vi "Tranfer String to Timestamp.vi"(9 "File Type":T1, 11 "String":string="44568.9754166667") -> (3 "time stamp":timestamp)   [LabVIEW 2020, in "Data Viewer.lvlib"]
uses:
  Data Viewer.lvlib
  File Type--enum.ctl
  <vilib>/Utility/miscctls.llb/LVDateTimeRec.ctl
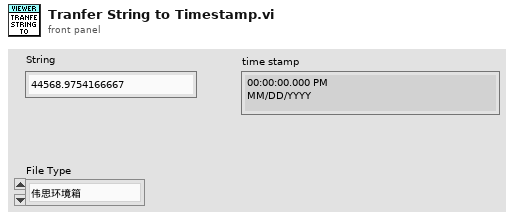
[diagram p1: front panel]
types:
  T1 = typedef "Data Viewer.lvlib/File Type--enum.ctl" = enum16{"伟思环境箱", "增达环境箱", "广五所环境箱", "无纸记录仪", "帕捷SA00339", "记录仪840", "记录仪8400", "记录仪MR888", "*.csv"}
  T2 = typedef "LVDateTimeRec.ctl" = cluster{"fractional second":dbl, "second":i32, "minute":i32, "hour":i32, "day of month":i32, "month":i32, "year":i32, "day of week":i32, "day of year":i32, "DST":i32}
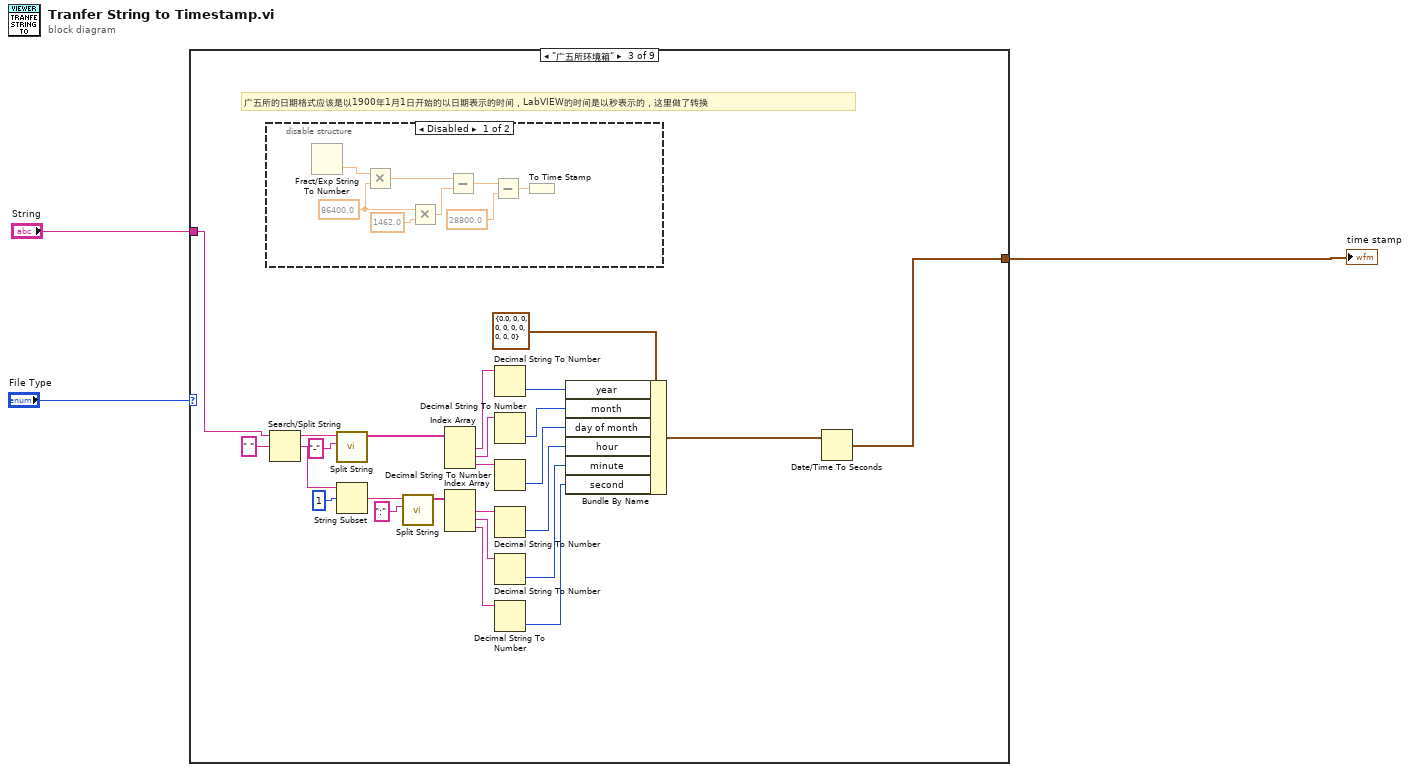
[diagram p0: block diagram]
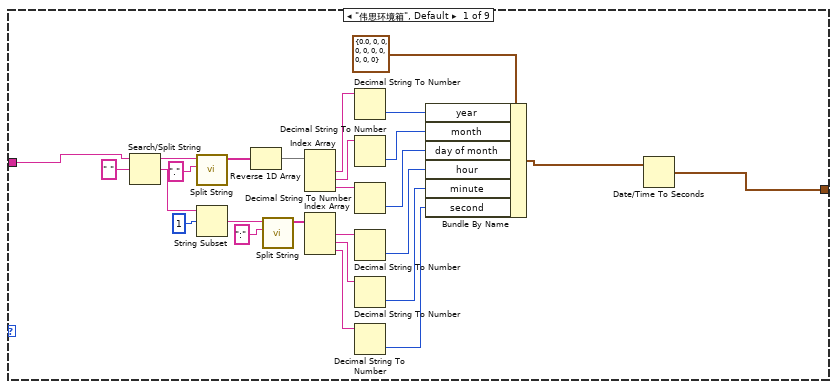
[diagram p2: hidden frame]
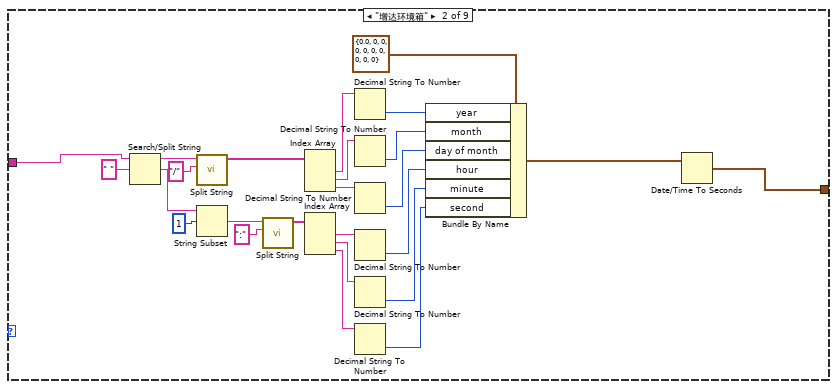
[diagram p3: hidden frame]
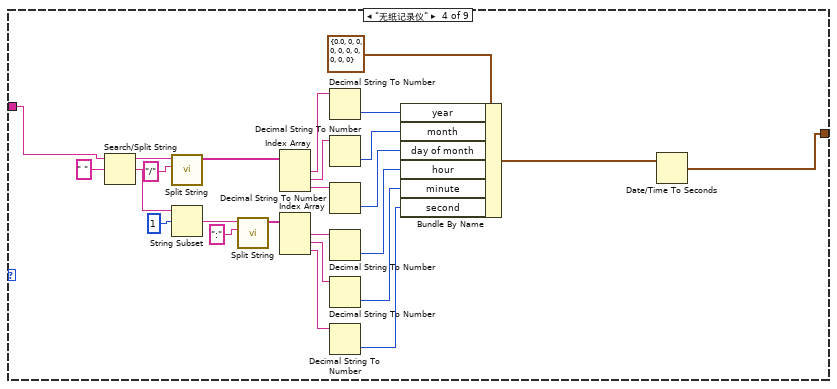
[diagram p5: hidden frame]
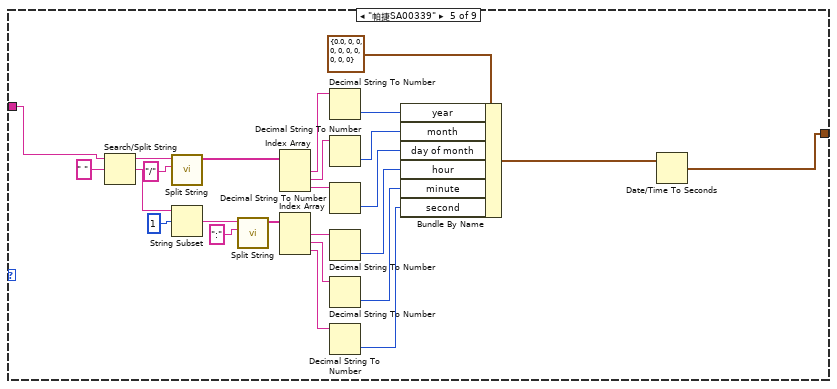
[diagram p6: hidden frame]
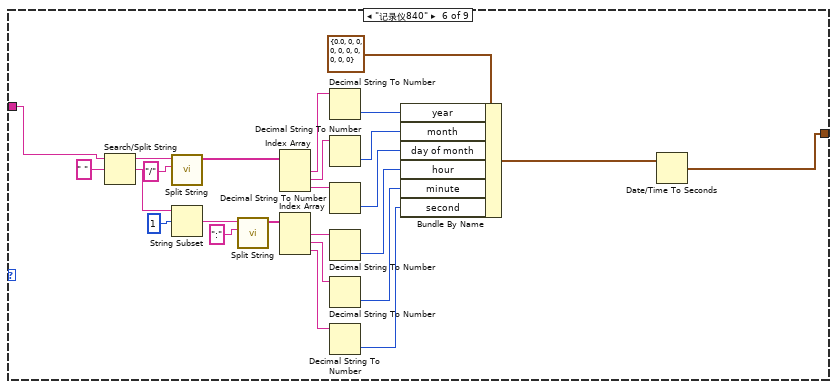
[diagram p7: hidden frame]
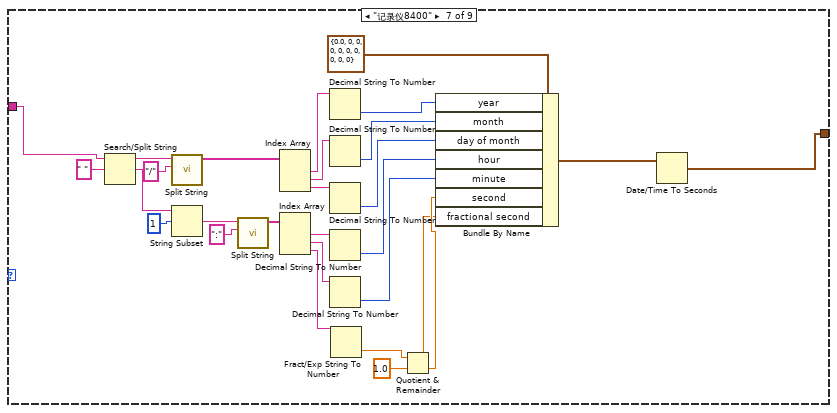
[diagram p8: hidden frame]
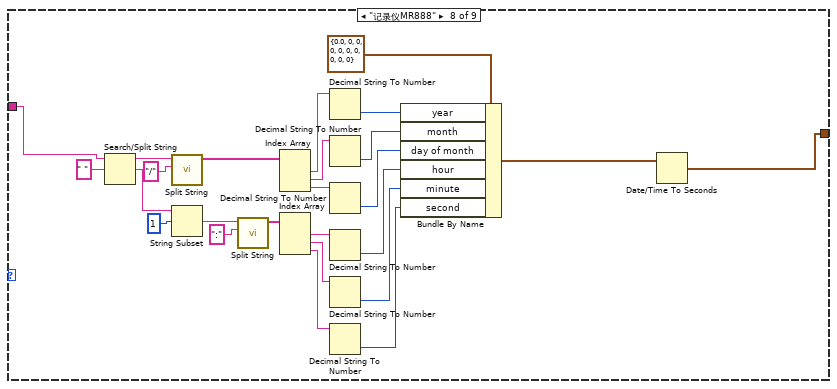
[diagram p9: hidden frame]
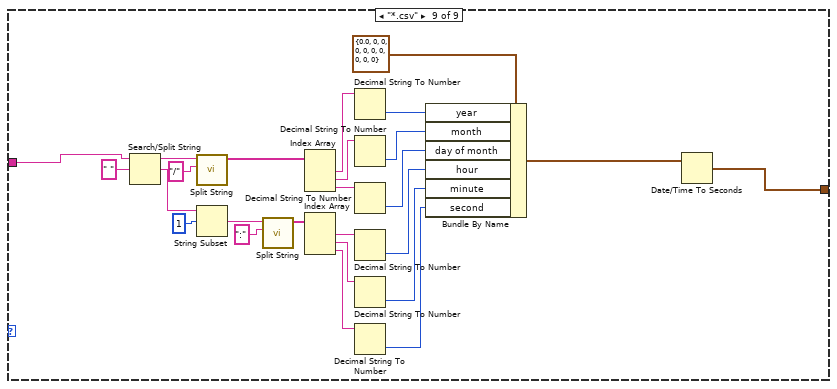
[diagram p10: hidden frame]
diagram:
  n1 = case shown="\"广五所环境箱\"" "File Type" {
    tunnel: "String" -> [w29 w54 w56 w112 w114 w139 w169 w192 w240]
    tunnel: [w4 w30 w55 w111 w113 w138 w168 w191 w216] -> w1
    frame "伟思环境箱", Default {
      n2 = Search/Split String(string=w29, search string/char (-)=" ") -> (substring before match=w22:string, match + rest of string=w27:string)  [unwired: 1 in, 1 out]
      n3 = call "Split String.vi"("分隔字符(;)"=".", "字符串"=w22) -> ("字符串数组"=w20:string[])  [unwired: 8 in, 1 out]
      n4 = String Subset(string=w27, offset (0)=1) -> (substring=w25:string)  [unwired: 1 in]
      n5 = Reverse 1D Array(array=w20) -> (reversed array=w19:string[])
      n6 = call "Split String.vi"("分隔字符(;)"=":", "字符串"=w25) -> ("字符串数组"=w9:string[])  [unwired: 8 in, 1 out]
      n7 = Index Array(array=w19) -> (element #1=w18:string, element #2=w17:string, element #3=w16:string)  [unwired: 3 in]
      n8 = Index Array(array=w9) -> (element #1=w10:string, element #2=w11:string, element #3=w12:string)  [unwired: 3 in]
      n9 = Decimal String To Number(string=w18) -> (number=w15:i32)  [unwired: 2 in, 1 out]
      n10 = Decimal String To Number(string=w17) -> (number=w14:i32)  [unwired: 2 in, 1 out]
      n11 = Decimal String To Number(string=w16) -> (number=w13:i32)  [unwired: 2 in, 1 out]
      n12 = Decimal String To Number(string=w10) -> (number=w7:i32)  [unwired: 2 in, 1 out]
      n13 = Decimal String To Number(string=w11) -> (number=w8:i32)  [unwired: 2 in, 1 out]
      n14 = Decimal String To Number(string=w12) -> (number=w6:i32)  [unwired: 2 in, 1 out]
      n15 = Bundle By Name(cluster=T2 {"fractional second"=0.0, "second"=0, "minute"=0, "hour"=0, "day of month"=0, "month"=0, "year"=0, "day of week"=0, "day of year"=0, "DST"=0} ("date time rec"), "year"=w15, "month"=w14, "day of month"=w13, "hour"=w7, "minute"=w8, "second"=w6) -> (w5:T2)
      n16 = Date/Time To Seconds(2:w5) -> (0:w4:timestamp)  [unwired: 1 in]
    }
    frame "增达环境箱" {
      n17 = Search/Split String(string=w54, search string/char (-)=" ") -> (substring before match=w47:string, match + rest of string=w52:string)  [unwired: 1 in, 1 out]
      n18 = call "Split String.vi"("分隔字符(;)"="/", "字符串"=w47) -> ("字符串数组"=w45:string[])  [unwired: 8 in, 1 out]
      n19 = String Subset(string=w52, offset (0)=1) -> (substring=w50:string)  [unwired: 1 in]
      n20 = call "Split String.vi"("分隔字符(;)"=":", "字符串"=w50) -> ("字符串数组"=w35:string[])  [unwired: 8 in, 1 out]
      n21 = Index Array(array=w45) -> (element #1=w44:string, element #2=w43:string, element #3=w42:string)  [unwired: 3 in]
      n22 = Index Array(array=w35) -> (element #1=w36:string, element #2=w37:string, element #3=w38:string)  [unwired: 3 in]
      n23 = Decimal String To Number(string=w44) -> (number=w41:i32)  [unwired: 2 in, 1 out]
      n24 = Decimal String To Number(string=w43) -> (number=w40:i32)  [unwired: 2 in, 1 out]
      n25 = Decimal String To Number(string=w42) -> (number=w39:i32)  [unwired: 2 in, 1 out]
      n26 = Decimal String To Number(string=w36) -> (number=w33:i32)  [unwired: 2 in, 1 out]
      n27 = Decimal String To Number(string=w37) -> (number=w34:i32)  [unwired: 2 in, 1 out]
      n28 = Decimal String To Number(string=w38) -> (number=w32:i32)  [unwired: 2 in, 1 out]
      n29 = Bundle By Name(cluster=T2 {"fractional second"=0.0, "second"=0, "minute"=0, "hour"=0, "day of month"=0, "month"=0, "year"=0, "day of week"=0, "day of year"=0, "DST"=0} ("date time rec"), "year"=w41, "month"=w40, "day of month"=w39, "hour"=w33, "minute"=w34, "second"=w32) -> (w31:T2)
      n30 = Date/Time To Seconds(2:w31) -> (0:w30:timestamp)  [unwired: 1 in]
    }
    frame "广五所环境箱" {
      # "广五所的日期格式应该是以1900年1月1日开始的以日期表示的时间，LabVIEW的时间是以秒表示的，这里做了转换"
      n31 = disable-structure shown="Disabled" {
        frame Disabled {
          w85 = 86400.0 ("y")
          n32 = Fract/Exp String To Number() -> (number=w87:dbl)  [unwired: 4 in, 1 out]
          n33 = Multiply(x=w87, y=w85) -> (x*y=w86:dbl)
          n34 = Multiply(x=w85, y=1462.0) -> (x*y=w83:dbl)
          n35 = Subtract(x=w86, y=w83) -> (x-y=w82:dbl)
          n36 = Subtract(x=w82, y=28800.0) -> (x-y=w80:dbl)
          n37 = To Time Stamp(1:w80) -> ()  [unwired: 1 out]
        }
        frame Enabled {
        }
      }
      n38 = Search/Split String(string=w56, search string/char (-)=" ") -> (substring before match=w73:string, match + rest of string=w78:string)  [unwired: 1 in, 1 out]
      n39 = call "Split String.vi"("分隔字符(;)"="-", "字符串"=w73) -> ("字符串数组"=w71:string[])  [unwired: 8 in, 1 out]
      n40 = String Subset(string=w78, offset (0)=1) -> (substring=w76:string)  [unwired: 1 in]
      n41 = call "Split String.vi"("分隔字符(;)"=":", "字符串"=w76) -> ("字符串数组"=w61:string[])  [unwired: 8 in, 1 out]
      n42 = Index Array(array=w71) -> (element #1=w70:string, element #2=w69:string, element #3=w68:string)  [unwired: 3 in]
      n43 = Index Array(array=w61) -> (element #1=w62:string, element #2=w63:string, element #3=w64:string)  [unwired: 3 in]
      n44 = Decimal String To Number(string=w70) -> (number=w67:i32)  [unwired: 2 in, 1 out]
      n45 = Decimal String To Number(string=w69) -> (number=w66:i32)  [unwired: 2 in, 1 out]
      n46 = Decimal String To Number(string=w68) -> (number=w65:i32)  [unwired: 2 in, 1 out]
      n47 = Decimal String To Number(string=w62) -> (number=w59:i32)  [unwired: 2 in, 1 out]
      n48 = Decimal String To Number(string=w63) -> (number=w60:i32)  [unwired: 2 in, 1 out]
      n49 = Decimal String To Number(string=w64) -> (number=w58:i32)  [unwired: 2 in, 1 out]
      n50 = Bundle By Name(cluster=T2 {"fractional second"=0.0, "second"=0, "minute"=0, "hour"=0, "day of month"=0, "month"=0, "year"=0, "day of week"=0, "day of year"=0, "DST"=0} ("date time rec"), "year"=w67, "month"=w66, "day of month"=w65, "hour"=w59, "minute"=w60, "second"=w58) -> (w57:T2)
      n51 = Date/Time To Seconds(2:w57) -> (0:w55:timestamp)  [unwired: 1 in]
    }
    frame "无纸记录仪" {
      n52 = Search/Split String(string=w112, search string/char (-)=" ") -> (substring before match=w104:string, match + rest of string=w109:string)  [unwired: 1 in, 1 out]
      n53 = call "Split String.vi"("分隔字符(;)"="/", "字符串"=w104) -> ("字符串数组"=w102:string[])  [unwired: 8 in, 1 out]
      n54 = String Subset(string=w109, offset (0)=1) -> (substring=w107:string)  [unwired: 1 in]
      n55 = call "Split String.vi"("分隔字符(;)"=":", "字符串"=w107) -> ("字符串数组"=w92:string[])  [unwired: 8 in, 1 out]
      n56 = Index Array(array=w102) -> (element #1=w101:string, element #2=w100:string, element #3=w99:string)  [unwired: 3 in]
      n57 = Index Array(array=w92) -> (element #1=w93:string, element #2=w94:string, element #3=w95:string)  [unwired: 3 in]
      n58 = Decimal String To Number(string=w101) -> (number=w98:i32)  [unwired: 2 in, 1 out]
      n59 = Decimal String To Number(string=w100) -> (number=w97:i32)  [unwired: 2 in, 1 out]
      n60 = Decimal String To Number(string=w99) -> (number=w96:i32)  [unwired: 2 in, 1 out]
      n61 = Decimal String To Number(string=w93) -> (number=w90:i32)  [unwired: 2 in, 1 out]
      n62 = Decimal String To Number(string=w94) -> (number=w91:i32)  [unwired: 2 in, 1 out]
      n63 = Decimal String To Number(string=w95) -> (number=w89:i32)  [unwired: 2 in, 1 out]
      n64 = Bundle By Name(cluster=T2 {"fractional second"=0.0, "second"=0, "minute"=0, "hour"=0, "day of month"=0, "month"=0, "year"=0, "day of week"=0, "day of year"=0, "DST"=0} ("date time rec"), "year"=w98, "month"=w97, "day of month"=w96, "hour"=w90, "minute"=w91, "second"=w89) -> (w88:T2)
      n65 = Date/Time To Seconds(2:w88) -> (0:w111:timestamp)  [unwired: 1 in]
    }
    frame "帕捷SA00339" {
      n66 = Search/Split String(string=w114, search string/char (-)=" ") -> (substring before match=w131:string, match + rest of string=w136:string)  [unwired: 1 in, 1 out]
      n67 = call "Split String.vi"("分隔字符(;)"="/", "字符串"=w131) -> ("字符串数组"=w129:string[])  [unwired: 8 in, 1 out]
      n68 = String Subset(string=w136, offset (0)=1) -> (substring=w134:string)  [unwired: 1 in]
      n69 = call "Split String.vi"("分隔字符(;)"=":", "字符串"=w134) -> ("字符串数组"=w119:string[])  [unwired: 8 in, 1 out]
      n70 = Index Array(array=w129) -> (element #1=w128:string, element #2=w127:string, element #3=w126:string)  [unwired: 3 in]
      n71 = Index Array(array=w119) -> (element #1=w120:string, element #2=w121:string, element #3=w122:string)  [unwired: 3 in]
      n72 = Decimal String To Number(string=w128) -> (number=w125:i32)  [unwired: 2 in, 1 out]
      n73 = Decimal String To Number(string=w127) -> (number=w124:i32)  [unwired: 2 in, 1 out]
      n74 = Decimal String To Number(string=w126) -> (number=w123:i32)  [unwired: 2 in, 1 out]
      n75 = Decimal String To Number(string=w120) -> (number=w117:i32)  [unwired: 2 in, 1 out]
      n76 = Decimal String To Number(string=w121) -> (number=w118:i32)  [unwired: 2 in, 1 out]
      n77 = Decimal String To Number(string=w122) -> (number=w116:i32)  [unwired: 2 in, 1 out]
      n78 = Bundle By Name(cluster=T2 {"fractional second"=0.0, "second"=0, "minute"=0, "hour"=0, "day of month"=0, "month"=0, "year"=0, "day of week"=0, "day of year"=0, "DST"=0} ("date time rec"), "year"=w125, "month"=w124, "day of month"=w123, "hour"=w117, "minute"=w118, "second"=w116) -> (w115:T2)
      n79 = Date/Time To Seconds(2:w115) -> (0:w113:timestamp)  [unwired: 1 in]
    }
    frame "记录仪840" {
      n80 = Search/Split String(string=w139, search string/char (-)=" ") -> (substring before match=w156:string, match + rest of string=w161:string)  [unwired: 1 in, 1 out]
      n81 = call "Split String.vi"("分隔字符(;)"="/", "字符串"=w156) -> ("字符串数组"=w154:string[])  [unwired: 8 in, 1 out]
      n82 = String Subset(string=w161, offset (0)=1) -> (substring=w159:string)  [unwired: 1 in]
      n83 = call "Split String.vi"("分隔字符(;)"=":", "字符串"=w159) -> ("字符串数组"=w144:string[])  [unwired: 8 in, 1 out]
      n84 = Index Array(array=w154) -> (element #1=w153:string, element #2=w152:string, element #3=w151:string)  [unwired: 3 in]
      n85 = Index Array(array=w144) -> (element #1=w145:string, element #2=w146:string, element #3=w147:string)  [unwired: 3 in]
      n86 = Decimal String To Number(string=w153) -> (number=w150:i32)  [unwired: 2 in, 1 out]
      n87 = Decimal String To Number(string=w152) -> (number=w149:i32)  [unwired: 2 in, 1 out]
      n88 = Decimal String To Number(string=w151) -> (number=w148:i32)  [unwired: 2 in, 1 out]
      n89 = Decimal String To Number(string=w145) -> (number=w142:i32)  [unwired: 2 in, 1 out]
      n90 = Decimal String To Number(string=w146) -> (number=w143:i32)  [unwired: 2 in, 1 out]
      n91 = Decimal String To Number(string=w147) -> (number=w141:i32)  [unwired: 2 in, 1 out]
      n92 = Bundle By Name(cluster=T2 {"fractional second"=0.0, "second"=0, "minute"=0, "hour"=0, "day of month"=0, "month"=0, "year"=0, "day of week"=0, "day of year"=0, "DST"=0} ("date time rec"), "year"=w150, "month"=w149, "day of month"=w148, "hour"=w142, "minute"=w143, "second"=w141) -> (w140:T2)
      n93 = Date/Time To Seconds(2:w140) -> (0:w138:timestamp)  [unwired: 1 in]
    }
    frame "记录仪8400" {
      n94 = Search/Split String(string=w169, search string/char (-)=" ") -> (substring before match=w184:string, match + rest of string=w189:string)  [unwired: 1 in, 1 out]
      n95 = call "Split String.vi"("分隔字符(;)"="/", "字符串"=w184) -> ("字符串数组"=w182:string[])  [unwired: 8 in, 1 out]
      n96 = String Subset(string=w189, offset (0)=1) -> (substring=w187:string)  [unwired: 1 in]
      n97 = call "Split String.vi"("分隔字符(;)"=":", "字符串"=w187) -> ("字符串数组"=w173:string[])  [unwired: 8 in, 1 out]
      n98 = Index Array(array=w182) -> (element #1=w181:string, element #2=w180:string, element #3=w179:string)  [unwired: 3 in]
      n99 = Index Array(array=w173) -> (element #1=w174:string, element #2=w175:string, element #3=w167:string)  [unwired: 3 in]
      n100 = Decimal String To Number(string=w181) -> (number=w178:i32)  [unwired: 2 in, 1 out]
      n101 = Decimal String To Number(string=w180) -> (number=w177:i32)  [unwired: 2 in, 1 out]
      n102 = Decimal String To Number(string=w179) -> (number=w176:i32)  [unwired: 2 in, 1 out]
      n103 = Decimal String To Number(string=w174) -> (number=w171:i32)  [unwired: 2 in, 1 out]
      n104 = Decimal String To Number(string=w175) -> (number=w172:i32)  [unwired: 2 in, 1 out]
      n105 = Fract/Exp String To Number(string=w167) -> (number=w166:dbl)  [unwired: 3 in, 1 out]
      n106 = Quotient & Remainder(x=w166, y=1.0) -> (x-y*floor(x/y)=w163:dbl, floor(x/y)=w164:dbl)
      n107 = Bundle By Name(cluster=T2 {"fractional second"=0.0, "second"=0, "minute"=0, "hour"=0, "day of month"=0, "month"=0, "year"=0, "day of week"=0, "day of year"=0, "DST"=0} ("date time rec"), "year"=w178, "month"=w177, "day of month"=w176, "hour"=w171, "minute"=w172, "second"=w164, "fractional second"=w163) -> (w170:T2)
      n108 = Date/Time To Seconds(2:w170) -> (0:w168:timestamp)  [unwired: 1 in]
    }
    frame "记录仪MR888" {
      n109 = Search/Split String(string=w192, search string/char (-)=" ") -> (substring before match=w209:string, match + rest of string=w214:string)  [unwired: 1 in, 1 out]
      n110 = call "Split String.vi"("分隔字符(;)"="/", "字符串"=w209) -> ("字符串数组"=w207:string[])  [unwired: 8 in, 1 out]
      n111 = String Subset(string=w214, offset (0)=1) -> (substring=w212:string)  [unwired: 1 in]
      n112 = call "Split String.vi"("分隔字符(;)"=":", "字符串"=w212) -> ("字符串数组"=w197:string[])  [unwired: 8 in, 1 out]
      n113 = Index Array(array=w207) -> (element #1=w206:string, element #2=w205:string, element #3=w204:string)  [unwired: 3 in]
      n114 = Index Array(array=w197) -> (element #1=w198:string, element #2=w199:string, element #3=w200:string)  [unwired: 3 in]
      n115 = Decimal String To Number(string=w206) -> (number=w203:i32)  [unwired: 2 in, 1 out]
      n116 = Decimal String To Number(string=w205) -> (number=w202:i32)  [unwired: 2 in, 1 out]
      n117 = Decimal String To Number(string=w204) -> (number=w201:i32)  [unwired: 2 in, 1 out]
      n118 = Decimal String To Number(string=w198) -> (number=w195:i32)  [unwired: 2 in, 1 out]
      n119 = Decimal String To Number(string=w199) -> (number=w196:i32)  [unwired: 2 in, 1 out]
      n120 = Decimal String To Number(string=w200) -> (number=w194:i32)  [unwired: 2 in, 1 out]
      n121 = Bundle By Name(cluster=T2 {"fractional second"=0.0, "second"=0, "minute"=0, "hour"=0, "day of month"=0, "month"=0, "year"=0, "day of week"=0, "day of year"=0, "DST"=0} ("date time rec"), "year"=w203, "month"=w202, "day of month"=w201, "hour"=w195, "minute"=w196, "second"=w194) -> (w193:T2)
      n122 = Date/Time To Seconds(2:w193) -> (0:w191:timestamp)  [unwired: 1 in]
    }
    frame "*.csv" {
      n123 = Search/Split String(string=w240, search string/char (-)=" ") -> (substring before match=w233:string, match + rest of string=w238:string)  [unwired: 1 in, 1 out]
      n124 = call "Split String.vi"("分隔字符(;)"="/", "字符串"=w233) -> ("字符串数组"=w231:string[])  [unwired: 8 in, 1 out]
      n125 = String Subset(string=w238, offset (0)=1) -> (substring=w236:string)  [unwired: 1 in]
      n126 = call "Split String.vi"("分隔字符(;)"=":", "字符串"=w236) -> ("字符串数组"=w221:string[])  [unwired: 8 in, 1 out]
      n127 = Index Array(array=w231) -> (element #1=w230:string, element #2=w229:string, element #3=w228:string)  [unwired: 3 in]
      n128 = Index Array(array=w221) -> (element #1=w222:string, element #2=w223:string, element #3=w224:string)  [unwired: 3 in]
      n129 = Decimal String To Number(string=w230) -> (number=w227:i32)  [unwired: 2 in, 1 out]
      n130 = Decimal String To Number(string=w229) -> (number=w226:i32)  [unwired: 2 in, 1 out]
      n131 = Decimal String To Number(string=w228) -> (number=w225:i32)  [unwired: 2 in, 1 out]
      n132 = Decimal String To Number(string=w222) -> (number=w219:i32)  [unwired: 2 in, 1 out]
      n133 = Decimal String To Number(string=w223) -> (number=w220:i32)  [unwired: 2 in, 1 out]
      n134 = Decimal String To Number(string=w224) -> (number=w218:i32)  [unwired: 2 in, 1 out]
      n135 = Bundle By Name(cluster=T2 {"fractional second"=0.0, "second"=0, "minute"=0, "hour"=0, "day of month"=0, "month"=0, "year"=0, "day of week"=0, "day of year"=0, "DST"=0} ("date time rec"), "year"=w227, "month"=w226, "day of month"=w225, "hour"=w219, "minute"=w220, "second"=w218) -> (w217:T2)
      n136 = Date/Time To Seconds(2:w217) -> (0:w216:timestamp)  [unwired: 1 in]
    }
  }
  "time stamp" <- w1
